vi "Path_arr.vi"(7 "MJ":enum16{"R", "W"}(ring), 11 "Path-arr":path[](array[path])) -> (3 "Path-arr 2":path[](array[path]))   [LabVIEW 2025, in "Path_management.lvclass"]
uses:
  Path_management.lvclass
panel:
  # "看好了奥\n这个vi可不是动态分布的喔"
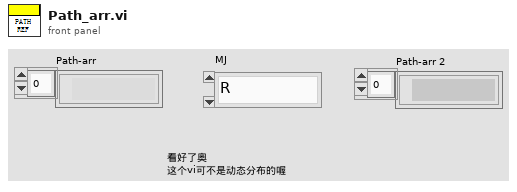
[diagram p1: front panel]
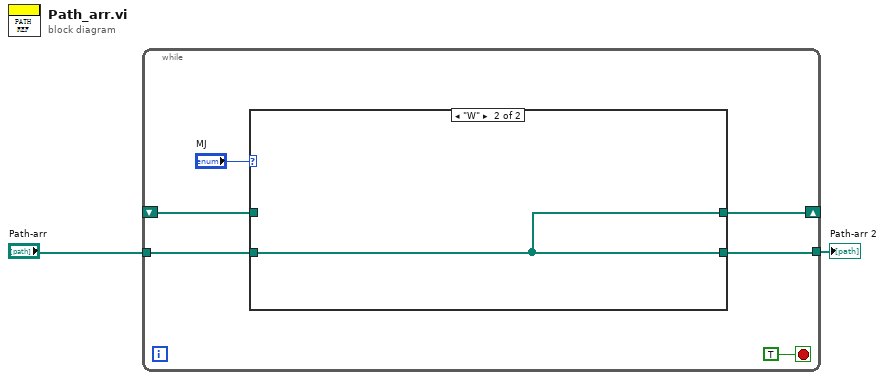
[diagram p0: block diagram]
diagram:
  n1 = while {
    shift-right: [w5] -> _
    shift-left: _ -> [w3]
    tunnel: "Path-arr" -> [w6]
    tunnel: [w4] -> w1
    stop <- TRUE stop-if-true
    n2 = case shown="\"W\"" "MJ" {
      tunnel: w6 -> [_ w10]
      tunnel: [w9 w10] -> w5
      tunnel: [w9 w10] -> w4
      tunnel: w3 -> [w9 _]
      frame "R", Default {
      }
      frame "W" {
      }
    }
  }
  "Path-arr 2" <- w1
